vi "Decode Received Data.vi"(11 "字符串输入":string) -> (2 "Data":string, 3 "Data Type":T1)   [LabVIEW 2020, in "TCP Communication.lvlib"]
uses:
  TCP Communication.lvlib
  Data Type.ctl
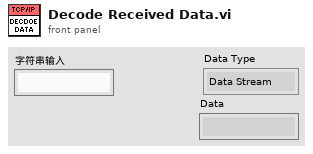
[diagram p1: front panel]
types:
  T1 = typedef "TCP Communication.lvlib/Data Type.ctl" = enum16{"Data Stream", "Status", "Request", "Reply"}
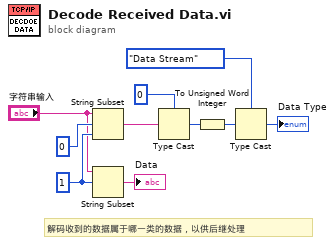
[diagram p0: block diagram]
diagram:
  w3 = 1 ("长度（剩余）")
  # "解码收到的数据属于哪一类的数据，以供后继处理"
  n1 = String Subset(string="字符串输入", offset (0)=0 ("偏移量(0)"), length (rest)=w3) -> (substring=w4:string)
  n2 = String Subset(string="字符串输入", offset (0)=w3) -> (substring=→"Data":string)  [unwired: 1 in]
  n3 = Type Cast(type=u8 0, x=w4) -> (*(type *) &x=w6:u8)
  n4 = To Unsigned Word Integer(number=w6) -> (unsigned 16bit integer=w7:u16)
  n5 = Type Cast(type=Data_Type."Data Stream" ("Data Type"), x=w7) -> (*(type *) &x=→"Data Type":T1)
